vi "Update Value.vi"(6 "Time":dbl, 8 "error in (no error)":errorcluster, 11 "ButtonControl in":refnum<class "DigitalButtonControl.lvclass">) -> (0 "error out":errorcluster, 1 "Update":bool, 2 "Value":variant, 3 "ButtonControl out":refnum<class "DigitalButtonControl.lvclass">)   [LabVIEW 2020, in "VolatusGUIElements.lvlib" / "DigitalButtonControl.lvclass"]
uses:
  DigitalButtonControl.lvclass
  DigitalButtonControl.lvclass/DigitalButtonControl.ctl
  lv-vecto/Vecto/Channel DBL/Channel DBL.lvclass/Channel DBL.ctl
  lv-vecto/Vecto/Group DBL/Value by Index.vi
  lv-vecto/Vecto/Channel DBL/Channel DBL.lvclass
  VolatusGUIElements.lvlib
  lv-vecto/Vecto/Vecto.lvlib
  VolatusGUI/Element Inhibit/Element Inhibit.lvclass
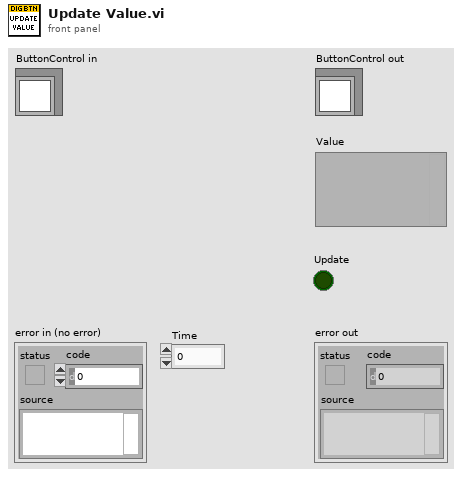
[diagram p1: front panel]
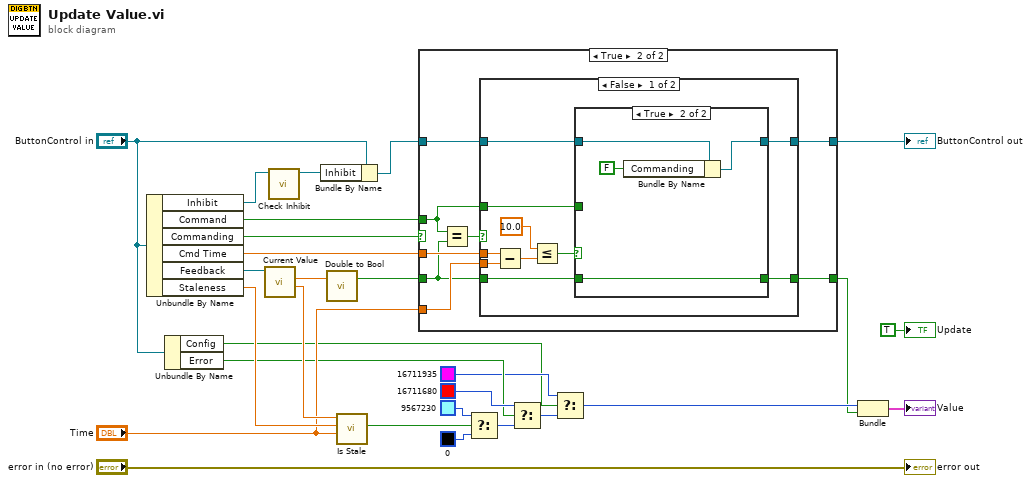
[diagram p0: block diagram]
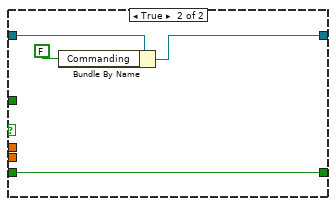
[diagram p4: hidden frame]
diagram:
  n1 = Unbundle By Name("ButtonControl in") -> ("Inhibit"=w3:refnum<class "Element Inhibit.lvclass">, "Command"=w10:bool, "Commanding"=w24:bool, "Cmd Time"=w22:dbl, "Feedback"=w27:refnum<class "Channel DBL.lvclass">, "Staleness"=w25:dbl)
  n2 = Unbundle By Name("ButtonControl in") -> ("Config"=w11:bool, "Error"=w14:bool)
  n3 = call "Current Value.vi"("Channel in"=w27) -> ("Timestamp"=w26:dbl, "Scaled"=w23:dbl)  [unwired: 6 in, 3 out]
  n4 = call "Check Inhibit.vi"("Element Inhibit in"=w3) -> ("Element Inhibit out"=w1:refnum<class "Element Inhibit.lvclass">)  [unwired: 9 in, 1 out]
  n5 = Bundle By Name(cluster="ButtonControl in", "Inhibit"=w1) -> (w2:refnum<class "DigitalButtonControl.lvclass">)
  n6 = call "Double to Bool.vi"("Double"=w23) -> ("Bool"=w21:bool)  [unwired: 2 in]
  n7 = call "Is Stale.vi"("Time"="Time", "Staleness"=w25, "Timestamp"=w26) -> ("Stale"=w19:bool)  [unwired: 8 in]
  n8 = case shown="True" w24 {
    tunnel: w21 -> [w30 w35]
    tunnel: w22 -> [_ w38]
    tunnel: "Time" -> [_ w37]
    tunnel: w10 -> [_ w31]
    tunnel: w2 -> [w29 w34]
    tunnel: [w29 w33] -> w8
    tunnel: [w30 w32] -> w6
    frame False {
    }
    frame True {
      n9 = Equal?(x=w31, y=w35) -> (x = y?=w36:bool)
      n10 = case shown="False" w36 {
        tunnel: w38 -> [w48 _]
        tunnel: w37 -> [w47 _]
        tunnel: w35 -> [w41 w55]
        tunnel: w34 -> [w43 w58]
        tunnel: [w42 w56] -> w33
        tunnel: [w39 w55] -> w32
        tunnel: w31 -> [w40 _]
        frame False {
          n11 = Subtract(x=w48, y=w47) -> (x-y=w46:dbl)
          n12 = Less Or Equal?(x=10.0, y=w46) -> (x <= y?=w44:bool)
          n13 = case shown="True" w44 {
            tunnel: w43 -> [w49 w54]
            tunnel: [w49 w52] -> w42
            tunnel: w41 -> [_ w51]
            tunnel: w40 -> [w50 _]
            tunnel: [w50 w51] -> w39
            frame False {
            }
            frame True {
              n14 = Bundle By Name(cluster=w54, "Commanding"=FALSE) -> (w52:refnum<class "DigitalButtonControl.lvclass">)
            }
          }
        }
        frame True {
          n15 = Bundle By Name(cluster=w58, "Commanding"=FALSE) -> (w56:refnum<class "DigitalButtonControl.lvclass">)
        }
      }
    }
  }
  "ButtonControl out" <- w8
  n16 = Select(t=u32 9567230, s=w19, f=u32 0) -> (s? t:f=w16:u32)
  n17 = Select(t=u32 16711680, s=w14, f=w16) -> (s? t:f=w13:u32)
  n18 = Select(t=u32 16711935, s=w11, f=w13) -> (s? t:f=w7:u32)
  n19 = Bundle(w7, "Bool"=w6) -> (→"Value":cluster{u32, "Bool":bool})  [unwired: 1 in]
  "error out" <- "error in (no error)"
  "Update" <- TRUE ("Update")
